vi "SlewRateLimiter_GetRate.vi"(11 "in SLEW_RATE_LIMITER":T1 {"NegativeRateLimit" format="%13.5p"; "PrevTime" format="%30.5p"; "PrevValue" format="%13.5p"; "PositiveRateLimit" format="%13.5p"}) -> (1 "NegativeRate":dbl, 3 "PositiveRate":dbl)   [LabVIEW 2019, in "Trajectory_Library.lvlib"]
doc: "Gets the current rate limit value.\n\nInputs:\n - in Slew Rate Limiter -- The Slew Rate Limiter data cluster\n \nOutputs:\n - PositiveRate -- The current positive rate limit in units/second. This is expected to be >= 0.\n - NegativeRate -- This current negative rate limit in units/second. This is expected to be <= 0."
uses:
  Trajectory_Library.lvlib
  TypeDef/SLEW_RATE_LIMITER.ctl
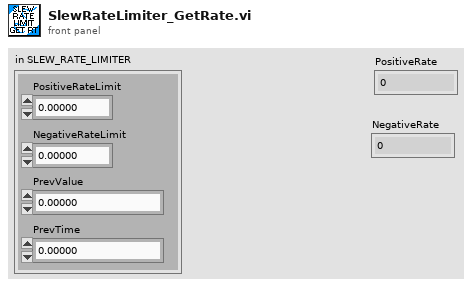
[diagram p1: front panel]
types:
  T1 = typedef "Trajectory_Library.lvlib/SLEW_RATE_LIMITER.ctl" = cluster{"PositiveRateLimit":dbl, "PrevValue":dbl, "PrevTime":dbl, "NegativeRateLimit":dbl}
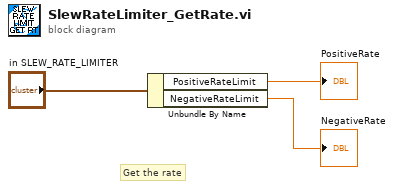
[diagram p0: block diagram]
diagram:
  # "Get the rate"
  n1 = Unbundle By Name("in SLEW_RATE_LIMITER") -> ("PositiveRateLimit"=→"PositiveRate":dbl, "NegativeRateLimit"=→"NegativeRate":dbl)
